vi "VIH - CHM Project - HHP Support - Close.vi"(8 "error in":errorcluster, 10 "write file (F)":bool, 11 "queue":T1) -> (0 "error out":errorcluster)   [LabVIEW 2014]
doc: "::: VI Helpeks :::\nCopyright (c) 2000-2026 Konstantin Shifershteyn. All rights reserved."
uses:
  VIH - CHM Project - HHP Support - Queue Refnum.ctl
  VIH - CHM Project - HHP Support - Config Data Cluster.ctl
panel:
  # "VI Helpeks\nCopyright (c) 2012-2026 Konstantin Shifershteyn"
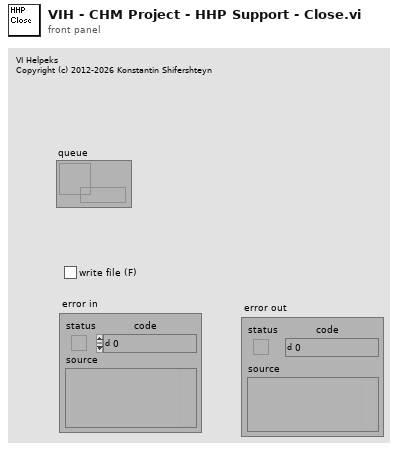
[diagram p1: front panel]
types:
  T1 = typedef "VIH - CHM Project - HHP Support - Queue Refnum.ctl" = refnum<queue>
  T2 = typedef "VIH - CHM Project - HHP Support - Config Data Cluster.ctl" = cluster{"Fille path":path, "sections":cluster{"Sec name":string, "key-values":string[][]}[]}
  T3 = cluster{"Sec name":string, "key-values":string[][]}[]
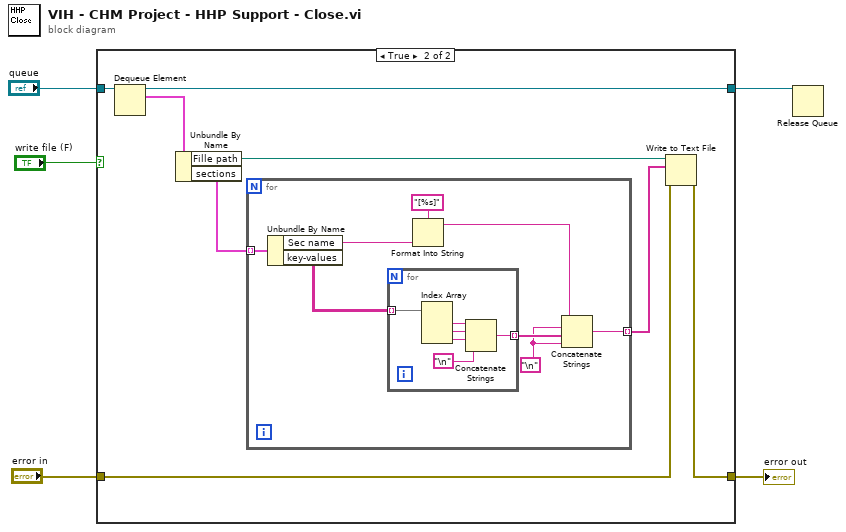
[diagram p0: block diagram]
diagram:
  n1 = case shown="True" "write file (F)" {
    tunnel: "queue" -> [w7 w15]
    tunnel: [w7 w10] -> w3
    tunnel: [w6 w8] -> w2
    tunnel: "error in" -> [w6 w9]
    frame False {
    }
    frame True {
      n2 = Dequeue Element(queue=w15) -> (queue out=w10:T1, element=w14:T2)  [unwired: 2 in, 2 out]
      n3 = Unbundle By Name(w14) -> ("Fille path"=w12:path, "sections"=w13:T3)
      n4 = for {
        tunnel: w13 -> [w23] mode=indexing
        tunnel: [w19] -> w11 mode=indexing
        w20 = "\n"
        n5 = Unbundle By Name(w23) -> ("Sec name"=w18:string, "key-values"=w22:string[][])
        n6 = for {
          tunnel: w22 -> [w29] mode=indexing
          tunnel: [w24] -> w21 mode=indexing
          n7 = Index Array(array=w29) -> (element #1=w28:string, element #2=w27:string, element #3=w26:string)  [unwired: 3 in]
          n8 = Concatenate Strings(w28, w27, w26, "\n") -> (w24:string)
        }
        n9 = Format Into String(format string="[%s]", w18) -> (resulting string=w16:string)  [unwired: 2 in, 1 out]
        n10 = Concatenate Strings(w16, w20, w21, w20) -> (w19:string)
      }
      n11 = Write to Text File(file (use dialog)=w12, text=w11, error in=w9) -> (error out=w8:errorcluster)  [unwired: 1 in, 2 out]
    }
  }
  "error out" <- w2
  n12 = Release Queue(queue=w3) -> ()  [unwired: 2 in, 3 out]
